vi "VIH Utility - MENU - Parse Menu String to Item Descriptors.vi"(8 "error in":errorcluster, 9 "comment sign ( // )":string="//", 10 "delimiter ( | )":string="|", 11 "Menu Description":string) -> (0 "error out":errorcluster, 2 "Item Descriptors":T1[](array[typedef]))   [LabVIEW 2014]
doc: "::: VI Helpeks :::\nCopyright (c) 2000-2026 Konstantin Shifershteyn. All rights reserved."
uses:
  VIH Utility - MENU - Menu Item Descriptor.ctl
  VIH Utility - MENU - Menu Item Type.ctl
panel:
  # "VI Helpeks\nCopyright (c) 2012-2026 Konstantin Shifershteyn"
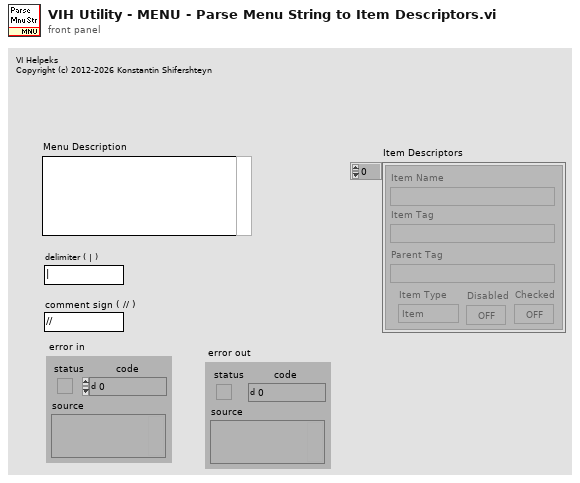
[diagram p1: front panel]
types:
  T1 = typedef "VIH Utility - MENU - Menu Item Descriptor.ctl" = cluster{"Item Name":string, "Item Tag":string, "Parent Tag":string, "Item Type":T2, "Disabled":bool, "Checked":bool}
  T2 = typedef "VIH Utility - MENU - Menu Item Type.ctl" = enum32{"Item", "SubMenu", "Separator"}
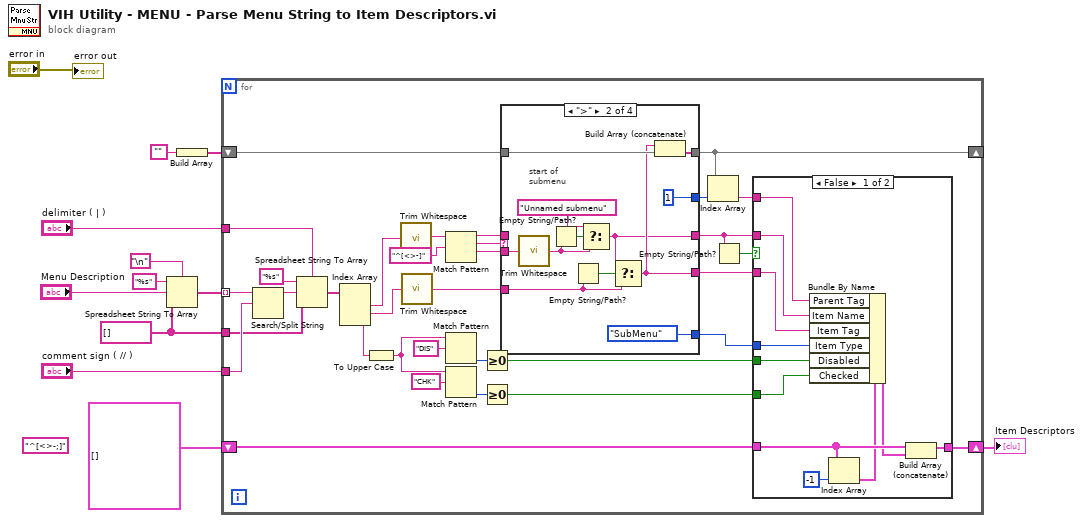
[diagram p0: block diagram]
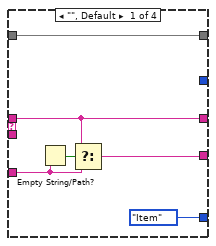
[diagram p3: hidden frame]
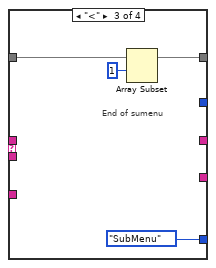
[diagram p4: hidden frame]
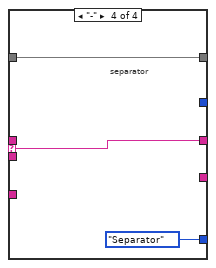
[diagram p5: hidden frame]
diagram:
  (unwired) "^[<>-;]" ("regular expression")
  w3 = string[] []
  n1 = Spreadsheet String To Array(delimiter (Tab)="\n", format string="%s", spreadsheet string="Menu Description", array type (2D Dbl)=w3) -> (array=w7:string[])
  n2 = Build Array("") -> (w9:string[])
  n3 = for {
    shift-right: [w32] -> _
    shift-left: w9 -> [w31]
    tunnel: w7 -> [w20] mode=indexing
    shift-right: [w29] -> w12
    shift-left: T1[] [] ("item descriptors") -> [w30]
    tunnel: "comment sign ( // )" -> [w19]
    tunnel: w3 -> [w17]
    tunnel: "delimiter ( | )" -> [w14]
    n4 = Search/Split String(string=w20, search string/char (-)=w19) -> (substring before match=w18:string)  [unwired: 3 out]
    n5 = Spreadsheet String To Array(delimiter (Tab)=w14, format string="%s", spreadsheet string=w18, array type (2D Dbl)=w17) -> (array=w13:string[])
    n6 = Index Array(array=w13) -> (element #1=w21:string, element #2=w22:string, element #3=w23:string)  [unwired: 3 in]
    n7 = To Upper Case(1:w23) -> (0:w35:string)
    n8 = call <vilib>:"Trim Whitespace.vi"("string"=w21) -> ("trimmed string"=w25:string)  [unwired: 1 in]
    n9 = call <vilib>:"Trim Whitespace.vi"("string"=w22) -> ("trimmed string"=w24:string)  [unwired: 1 in]
    n10 = Match Pattern(string=w25, regular expression="^[<>-]") -> (before substring=w43:string, match substring=w45:string, after substring=w44:string)  [unwired: 2 out]
    n11 = Match Pattern(string=w35, regular expression="DIS") -> (offset past match=w37:i32)  [unwired: 4 out]
    n12 = Match Pattern(string=w35, regular expression="CHK") -> (offset past match=w39:i32)  [unwired: 4 out]
    n13 = Greater Or Equal To 0?(x=w37) -> (x >= 0?=w33:bool)
    n14 = Greater Or Equal To 0?(x=w39) -> (x >= 0?=w34:bool)
    n15 = case shown="\">\"" w45 {
      selector: w45 -> [_ _ _ w82]
      tunnel: w31 -> [w63 w74 w77 w81]
      tunnel: w44 -> [_ w72 _ _]
      tunnel: [w63 w75 w78 w81] -> w32
      tunnel: [w61 w65 _ w82] -> w26
      tunnel: w43 -> [w61 _ _ _]
      tunnel: [w58 w69 _ _] -> w42
      tunnel: [_ 1 _ _] -> w40
      tunnel: w24 -> [w62 w70 _ _]
      tunnel: [VIH_Utility_-_MENU_-_Menu_Item_Type."Item" ("Item Type") VIH_Utility_-_MENU_-_Menu_Item_Type."SubMenu" ("Item Type") VIH_Utility_-_MENU_-_Menu_Item_Type."SubMenu" ("Item Type") VIH_Utility_-_MENU_-_Menu_Item_Type."Separator" ("Item Type")] -> w28
      frame "", Default {
        n16 = Empty String/Path?(string/path=w62) -> (empty?=w59:bool)
        n17 = Select(t=w61, s=w59, f=w62) -> (s? t:f=w58:string)
      }
      frame ">" {
        # "start of\nsubmenu"
        n18 = call <vilib>:"Trim Whitespace.vi"("string"=w72) -> ("trimmed string"=w67:string)  [unwired: 1 in]
        n19 = Empty String/Path?(string/path=w67) -> (empty?=w66:bool)
        n20 = Empty String/Path?(string/path=w70) -> (empty?=w71:bool)
        n21 = Select(t="Unnamed submenu", s=w66, f=w67) -> (s? t:f=w65:string)
        n22 = Select(t=w65, s=w71, f=w70) -> (s? t:f=w69:string)
        n23 = Build Array (concatenate)(w69, w74) -> (w75:string[])
      }
      frame "<" {
        # "End of sumenu"
        n24 = Array Subset(array=w77, index=1) -> (w78:string[])  [unwired: 1 in]
      }
      frame "-" {
        # "separator"
      }
    }
    n25 = Index Array(array=w32, index=w40) -> (element=w41:string)
    n26 = Empty String/Path?(string/path=w26) -> (empty?=w27:bool)
    n27 = case shown="False" w27 {
      tunnel: w26 -> [w51 _]
      tunnel: w42 -> [w46 _]
      tunnel: w41 -> [w50 _]
      tunnel: w34 -> [w48 _]
      tunnel: w33 -> [w49 _]
      tunnel: w30 -> [w55 w57]
      tunnel: [w56 w57] -> w29
      tunnel: w28 -> [w47 _]
      frame False {
        n28 = Index Array(array=w55, index=-1) -> (element=w53:T1)
        n29 = Bundle By Name(cluster=w53, "Parent Tag"=w50, "Item Name"=w51, "Item Tag"=w46, "Item Type"=w47, "Disabled"=w49, "Checked"=w48) -> (w52:T1)
        n30 = Build Array (concatenate)(w55, w52) -> (w56:T1[])
      }
      frame True {
      }
    }
  }
  "Item Descriptors" <- w12
  "error out" <- "error in"
